vi "CSE ISP - pre-execution operations.vi"(6 "run specs":T2 {"Run mode" items=["Regular", "Debugging", "Callback VI"]}, 8 "directives":T1={"enaNamedConst"=TRUE}, 9 "script":string, 10 "item subtag":string, 11 "ISP menu":refnum<k9>) -> (0 "error out":errorcluster, 1 "exec params":T6={"pause counter"=1000, "pause, ms"=0, "autoVar"=TRUE, "enCpx"=TRUE}, 2 "Callback VI RefNum":T3, 3 "CSE RefNum":T5, 4 "test syntax only":bool, 5 "VC Handle":T4=-1, 7 "loaded functions":string[](array[string]))   [LabVIEW 2021]
doc: "::: CalcExpress Toolkit :::\nCopyright (c) 2000-2026 Konstantin Shifershteyn. All rights reserved."
uses:
  vi.lib/addons/CalcExpress/cse.llb/CSE Instance RefNum.ctl
  vi.lib/addons/CalcExpress/cetypes.llb/VarMan Variable Context Handle.ctl
  vi.lib/addons/CalcExpress/cse.llb/CSE Callback VI RefNum.ctl
  vi.lib/addons/CalcExpress/cetypes.llb/CSE Parsing Directives.ctl
  vi.lib/addons/CalcExpress/cse.llb/CSE Type - Callback Call Reason.ctl
panel:
  # "This VI has to be reentrant in order\nto provide more than one CSE ISP\ninstances are running at a time"
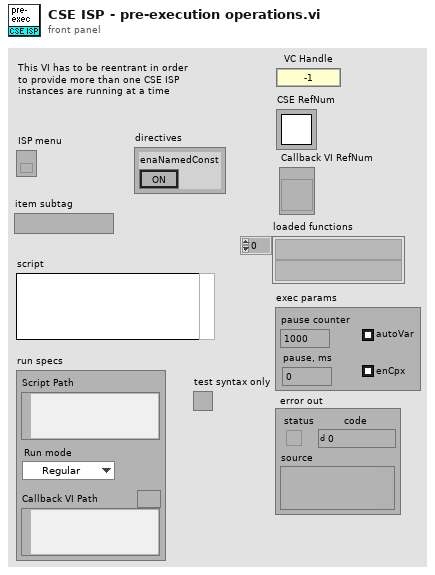
[diagram p1: front panel]
types:
  T1 = typedef "CSE Parsing Directives.ctl" = cluster{"enaNamedConst":bool}
  T2 = cluster{"Script Path":path, "Run mode":u32, "Callback VI Path":path}
  T3 = typedef "CSE Callback VI RefNum.ctl" = refnum<vi>
  T4 = typedef "VarMan Variable Context Handle.ctl" = i32
  T5 = typedef "CSE Instance RefNum.ctl" = refnum<k1>
  T6 = cluster{"pause counter":i32, "pause, ms":i32, "autoVar":bool, "enCpx":bool}
  T7 = cluster{"reuse context":bool, "reuse variables":bool, "keep variables":bool}
  T8 = cluster{"AutoParse":bool, "GroupStm":bool, "ErrSrcMaxLen":i32}
  T9 = cluster{"unload FuncVIs":bool, "debug: line mode":bool}
  T10 = typedef "CSE Type - Callback Call Reason.ctl" = u32
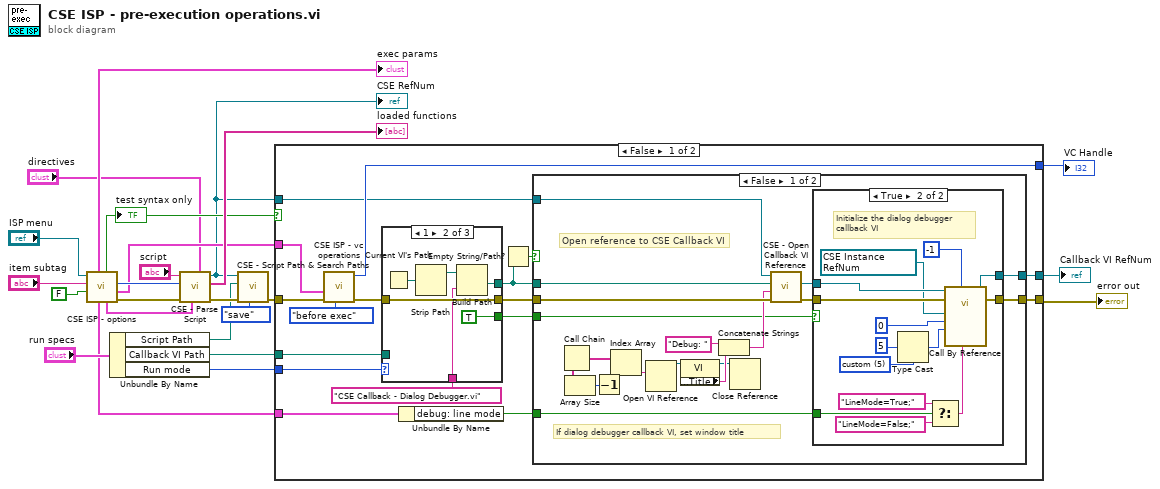
[diagram p0: block diagram]
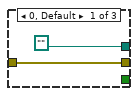
[diagram p2: hidden frame]
diagram:
  n1 = call "CSE ISP - options.vi"("enable menu (T)"=FALSE, "item subtag"="item subtag", "ISP menu"="ISP menu") -> ("error out"=w13:errorcluster, "VM params"=w15:T7, "load FuncVIs"=w22:u32, "Parse params"=w23:T8, "test syntax only"=w17:bool, "misc params"=w8:T9, "Exec params"=→"exec params":T6)  [unwired: 1 in, 1 out]
  "test syntax only" <- w17
  n2 = Unbundle By Name("run specs") -> ("Script Path"=w3:path, "Callback VI Path"=w10:path, "Run mode"=w11:u32)
  n3 = call "CSE - Parse Script.vi"("directives"="directives", "parameters"=w23, "error in"=w13, "load FuncVIs"=w22, "Script"="script") -> ("error out"=w6:errorcluster, "loaded functions"=→"loaded functions":string[], "CSE RefNum"=w5:T5)  [unwired: 2 in, 2 out]
  "CSE RefNum" <- w5
  n4 = call "CSE - Script Path & Search Paths.vi"("action"=enum32{"get", "save"}."save", "error in"=w6, "script file path"=w3, "CSE RefNum"=w5) -> ("error out"=w7:errorcluster)  [unwired: 4 in, 3 out]
  n5 = case shown="False" w17 {
    tunnel: w7 -> [w41 w87]
    tunnel: [w33 w87] -> w9
    tunnel: [w40 _] -> w16
    tunnel: w15 -> [w39 _]
    tunnel: [w32 _] -> w2
    tunnel: w11 -> [w31 _]
    tunnel: w10 -> [w30 _]
    tunnel: w8 -> [w28 _]
    tunnel: w5 -> [w25 _]
    frame False {
      n6 = call "CSE ISP - vc operations.vi"("cmd"=enum16{"before exec", "after exec", "init"}."before exec", "error in"=w41, "params"=w39) -> ("error out"=w34:errorcluster, "VC Handle"=w40:T4)  [unwired: 7 in]
      n7 = case shown="1" w31 {
        tunnel: [w43 w49 w51] -> w35
        tunnel: w34 -> [w43 w49 w51]
        tunnel: [path "" w46 w50] -> w37
        tunnel: w30 -> [_ _ w50]
        tunnel: "CSE Callback - Dialog Debugger.vi" ("append path") -> [_ w45 _]
        tunnel: [_ TRUE _] -> w26
        frame 0, Default {
        }
        frame 1 {
          n8 = Current VI's Path() -> (path=w48:path)
          n9 = Strip Path(path=w48) -> (stripped path=w47:path)  [unwired: 1 out]
          n10 = Build Path(base path=w47, name or relative path=w45) -> (appended path=w46:path)
        }
        frame 2 {
        }
      }
      n11 = Unbundle By Name(w28) -> ("debug: line mode"=w27:bool)
      n12 = Empty String/Path?(string/path=w37) -> (empty?=w36:bool)
      n13 = case shown="False" w36 {
        tunnel: w35 -> [w66 w86]
        tunnel: w37 -> [w65 _]
        tunnel: [w68 w86] -> w33
        tunnel: [w69 _] -> w32
        tunnel: w27 -> [w67 _]
        tunnel: w26 -> [w60 _]
        tunnel: w25 -> [w61 _]
        frame False {
          # "If dialog debugger callback VI, set window title"
          # "Open reference to CSE Callback VI"
          n14 = Call Chain() -> (call chain=w54:string[])
          n15 = Array Size(array=w54) -> (size(s)=w52:i32)
          n16 = Decrement(x=w52) -> (x-1=w53:i32)
          n17 = Index Array(array=w54, index=w53) -> (element=w55:string)
          n18 = Open VI Reference(vi path=w55) -> (vi reference=w56:refnum<vi>)  [unwired: 5 in, 1 out]
          n19 = property class="VI"(reference=w56) -> (reference out=w57:refnum<vi>, "Front Panel Window:Title"=w59:string)  [unwired: 1 in, 1 out]
          n20 = Concatenate Strings("Debug: " ("string"), w59) -> (w62:string)
          n21 = Close Reference(reference=w57) -> ()  [unwired: 1 in, 1 out]
          n22 = call "CSE - Open Callback VI Reference.vi"("error in"=w66, "Window Title"=w62, "Callback VI Path"=w65, "CSE RefNum"=w61) -> ("error out"=w63:errorcluster, "Callback VI RefNum"=w64:T3)  [unwired: 5 in, 1 out]
          n23 = case shown="True" w60 {
            tunnel: w63 -> [w71 w76]
            tunnel: [w70 w82] -> w69
            tunnel: [w71 w81] -> w68
            tunnel: w67 -> [_ w77]
            tunnel: w64 -> [w70 w75]
            frame False {
            }
            frame True {
              w72 = T5 refnum items=["CSE RefNum"] ("CSE RefNum")
              w83 = T10 5 items=["Exec Start", "Action completed", "pause to breath", "reserved 1", "reserved 2", "custom"] ("Call Reason")
              # "Initialize the dialog debugger\ncallback VI"
              n24 = Type Cast(type=w83, x=u32 5) -> (*(type *) &x=w84:T10)
              n25 = Select(t="LineMode=True;" ("string (\"\")"), s=w77, f="LineMode=False;" ("string (\"\")")) -> (s? t:f=w78:string)
              n26 = call-by-ref "?"(reference=w75, error in=w76, "Custom data"=w78, "VC Handle"=T4 -1, "Call Reason"=w84, "Stm Index"=0, "CSE RefNum"=w72) -> (reference out=w82:T3, error out=w81:errorcluster)  [unwired: 1 in, 6 out]
            }
          }
        }
        frame True {
        }
      }
    }
    frame True {
    }
  }
  "VC Handle" <- w16
  "error out" <- w9
  "Callback VI RefNum" <- w2
